vi "ZM-PC-getDataAsJson.vi"(8 "error in (no error)":errorcluster, 11 "ZM-PC-package in":refnum<class "ZM-PC-package.lvclass">) -> (0 "error out":errorcluster, 2 "json":string, 3 "ZM-PC-package out":refnum<class "ZM-PC-package.lvclass">)   [LabVIEW 2020, in "ZM-PC-packages.lvlib" / "ZM-PC-package.lvclass"]
doc: "Returns the package as one JSON object (dynamic dispatch). The parent flattens only the header from getHeader: {\"timestamp\":\"...\",\"type\":\"Undefined\",\"destination\":\"Unknown\"}, LabVIEW JSON extensions off. Each child overrides it with its own body (header plus data)."
uses:
  ZM-PC-package.lvclass
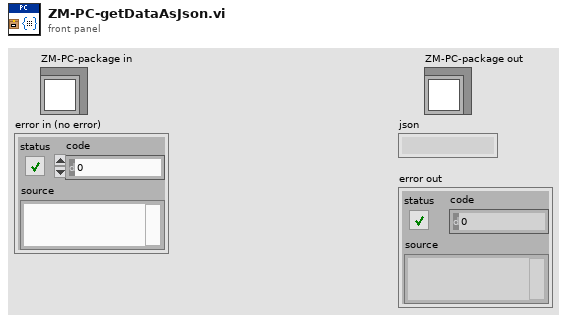
[diagram p1: front panel]
types:
  T1 = typedef "ZM-PC-packages.lvlib/ZM-PC-package.lvclass/ZM-PC-HEADER.ctl" = cluster{"timestamp":string, "type":string, "destination":string}
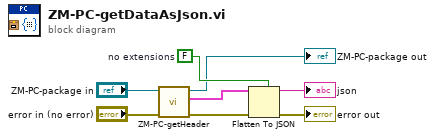
[diagram p0: block diagram]
diagram:
  w4 = FALSE  # no extensions
  n1 = call "ZM-PC-getHeader.vi"("error in (no error)"="error in (no error)", "ZM-PC-package in"="ZM-PC-package in") -> ("error out"=w5:errorcluster, "header"=w6:T1, "ZM-PC-package out"=→"ZM-PC-package out":refnum<class "ZM-PC-package.lvclass">)  [unwired: 7 in]
  n2 = Flatten To JSON(enable LabVIEW extensions? (T)=w4, anything=w6, error in (no error)=w5) -> (JSON string=→"json":string, 11:→"error out":errorcluster)
